vi "GenerateHTML.vi"(6 "Unattended Mode":bool, 8 "error in (no error)":errorcluster, 9 "Files to preload":path[](array[path]), 10 "Destination Directory":path, 11 "Source directory/files":path) -> (0 "error out":errorcluster, 3 "Output":string)   [LabVIEW 2017]
uses:
  JsonConverters/ConverterBase/FileConverterBase.lvclass
  JsonConverters/LVFileConverters/ClassConverter/ClassConverter.lvclass
  C:/FINALE/src/HTMLGenerator/JsonConverters/ConverterBase/FileConverterBase.lvclass
  JsonConverters/LVFileConverters/VIConverter/VIConverter.lvclass
  PathConfiguration.vi
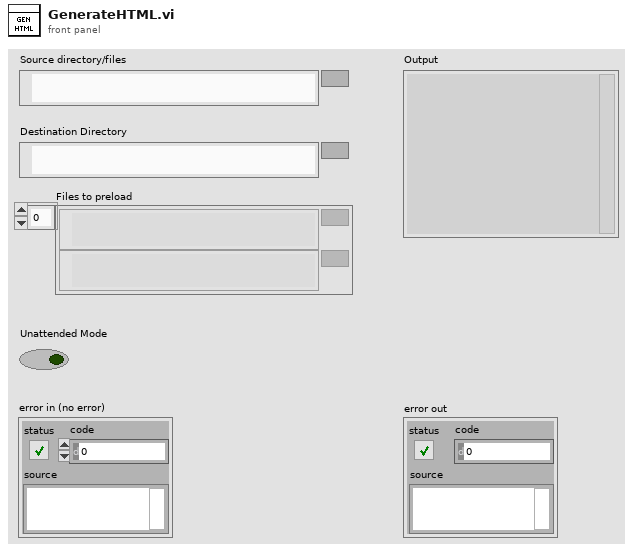
[diagram p1: front panel]
types:
  T1 = typedef "ApplicationItems.ctl" = cluster{"Application Reference":refnum<vi>, "Files":T2[]}
  T2 = typedef "SourceJsonPaths.ctl" = cluster{"File to convert":path, "Output directory":path}
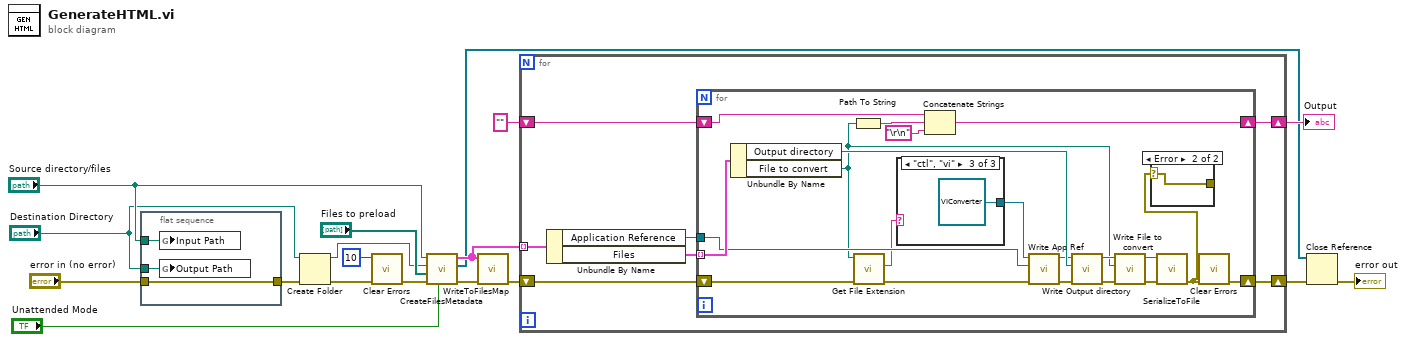
[diagram p0: block diagram]
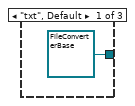
[diagram p3: hidden frame]
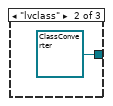
[diagram p4: hidden frame]
diagram:
  n1 = flat-sequence {
    tunnel: "Source directory/files" -> [w21]
    tunnel: "Destination Directory" -> [w20]
    tunnel: "error in (no error)" -> [w19]
    tunnel: [w19] -> w8
    frame #0 {
      n2 = global write "PathConfiguration.vi" "Input Path"(w21) -> ()
      n3 = global write "PathConfiguration.vi" "Output Path"(w20) -> ()
    }
  }
  n4 = Create Folder(path (use dialog)="Destination Directory", error in=w8) -> (created path=w9:path, error out=w7:errorcluster)  [unwired: 1 in, 1 out]
  n5 = call <vilib>:"Clear Errors.vi"("error in (no error)"=w7, "specific error code to clear (0: all)"=10) -> ("error out"=w6:errorcluster)  [unwired: 4 in, 1 out]
  n6 = call "CreateFilesMetadata.vi"("Unattended Mode"="Unattended Mode", "error in (no error)"=w6, "Files to preload"="Files to preload", "Output Directory"=w9, "Source directory/files"="Source directory/files") -> ("error out"=w14:errorcluster, "Opened file refs"=w2:refnum<vi>[], "Items To Serialize"=w12:T1[])  [unwired: 4 in]
  n7 = call "WriteToFilesMap.vi"("error in (no error)"=w14, "Items To Serialize"=w12) -> ("error out"=w13:errorcluster)  [unwired: 9 in]
  n8 = for {
    shift-right: [w27] -> w4
    shift-left: w13 -> [w28]
    tunnel: w12 -> [w26] mode=indexing
    shift-right: [w24] -> w15
    shift-left: "" -> [w22]
    n9 = Unbundle By Name(w26) -> ("Application Reference"=w25:refnum<vi>, "Files"=w23:T2[])
    n10 = for {
      tunnel: w25 -> [w39]
      tunnel: w23 -> [w40] mode=indexing
      shift-right: [w30] -> w27
      shift-left: w28 -> [w37]
      shift-right: [w33] -> w24
      shift-left: w22 -> [w35]
      n11 = Unbundle By Name(w40) -> ("Output directory"=w48:path, "File to convert"=w34:path)
      n12 = Path To String(path=w34) -> (string=w32:string)
      n13 = call <vilib>:"Get File Extension.vi"("error in (no error)"=w37, "file"=w34) -> ("error out"=w36:errorcluster, "lowercase file extension"=w38:string)  [unwired: 5 in, 3 out]
      n14 = case shown="\"ctl\", \"vi\"" w38 {
        tunnel: [refnum<class "FileConverterBase.lvclass"> refnum ("FileConverterBase.lvclass") refnum<class "ClassConverter.lvclass"> refnum ("ClassConverter.lvclass") refnum<class "VIConverter.lvclass"> refnum ("VIConverter.lvclass")] -> w47
        frame "txt", Default {
        }
        frame "lvclass" {
        }
        frame "ctl", "vi" {
        }
      }
      n15 = Concatenate Strings(w35, w32, "\r\n") -> (w33:string)
      n16 = call-dynamic "Write App Ref.vi"("error in (no error)"=w36, "App Ref"=w39, "FileConverterBase in"=w47) -> ("error out"=w41:errorcluster, "FileConverterBase out"=w46:refnum<class "FileConverterBase.lvclass">)  [unwired: 7 in]
      n17 = call-dynamic "Write Output directory.vi"("error in (no error)"=w41, "Output JSON File Path"=w48, "FileConverterBase in"=w46) -> ("error out"=w42:errorcluster, "FileConverterBase out"=w45:refnum<class "FileConverterBase.lvclass">)  [unwired: 7 in]
      n18 = call-dynamic "Write File to convert.vi"("error in (no error)"=w42, "Input File Path"=w34, "FileConverterBase in"=w45) -> ("error out"=w43:errorcluster, "FileConverterBase out"=w44:refnum<class "FileConverterBase.lvclass">)  [unwired: 7 in]
      n19 = call-dynamic "SerializeToFile.vi"("error in (no error)"=w43, "FileConverterBase in"=w44) -> ("error out"=w29:errorcluster)  [unwired: 8 in, 1 out]
      n20 = case shown="Error" w29 {
        selector: w29 -> [w49 w50]
        tunnel: [w49 w50] -> _
        frame No Error {
        }
        frame Error {
        }
      }
      n21 = call <vilib>:"Clear Errors.vi"("error in (no error)"=w29) -> ("error out"=w30:errorcluster)  [unwired: 5 in, 1 out]
    }
  }
  "Output" <- w15
  n22 = Close Reference(reference=w2, error in (no error)=w4) -> (error out=→"error out":errorcluster)
